vi "resolve url.vi"(10 "provided path":string, 11 "Base URL":string) -> (3 "resolved url":string)   [LabVIEW 2020, in "reqwest.lvclass"]
uses:
  reqwest.lvclass
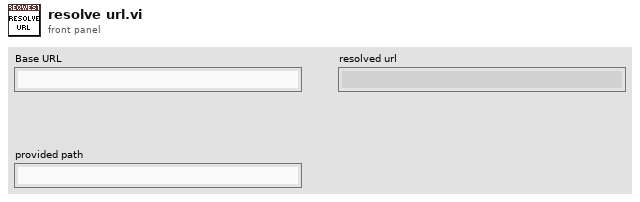
[diagram p1: front panel]
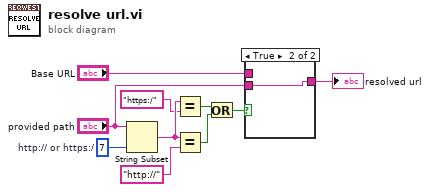
[diagram p0: block diagram]
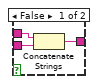
[diagram p2: hidden frame]
diagram:
  w8 = 7  # http:// or https:/
  n1 = String Subset(string="provided path", length (rest)=w8) -> (substring=w7:string)  [unwired: 1 in]
  n2 = Equal?(x=w7, y="https:/") -> (x = y?=w3:bool)
  n3 = Equal?(x=w7, y="http://") -> (x = y?=w4:bool)
  n4 = Or(x=w3, y=w4) -> (x .or. y?=w2:bool)
  n5 = case shown="True" w2 {
    tunnel: [w13 w14] -> w10
    tunnel: "Base URL" -> [w12 _]
    tunnel: "provided path" -> [w11 w14]
    frame False {
      n6 = Concatenate Strings(w12, w11) -> (w13:string)
    }
    frame True {
    }
  }
  "resolved url" <- w10
